vi "IR ini file file Read.vi"(2 "configuration file path":path, 11 "error in (no error) 2":errorcluster) -> (3 "IR Voltage":dbl, 4 "Ramp Time":dbl, 6 "IR LO SET resistance value(M£[)":u16=2 min=1 max=9999, 8 "IR Time":dbl, 10 "IR HI SET resistance value(M£[)":u16=9999 min=2 max=9999, 15 "error in (no error) 3":errorcluster)   [LabVIEW 2021]
uses:
  Template/Main_VI/Control/Ini.ctl
panel:
  # "M£["
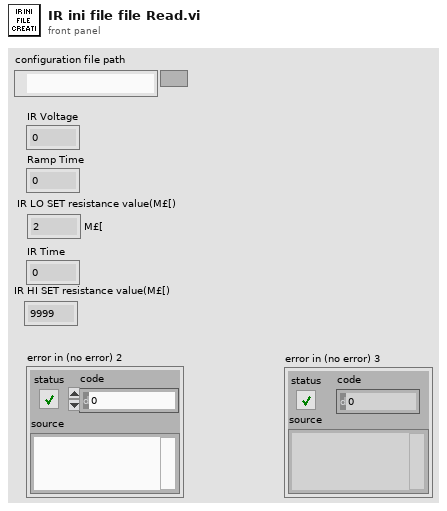
[diagram p1: front panel]
types:
  T1 = typedef "Ini.ctl" = enum16{"Write", "Read"}
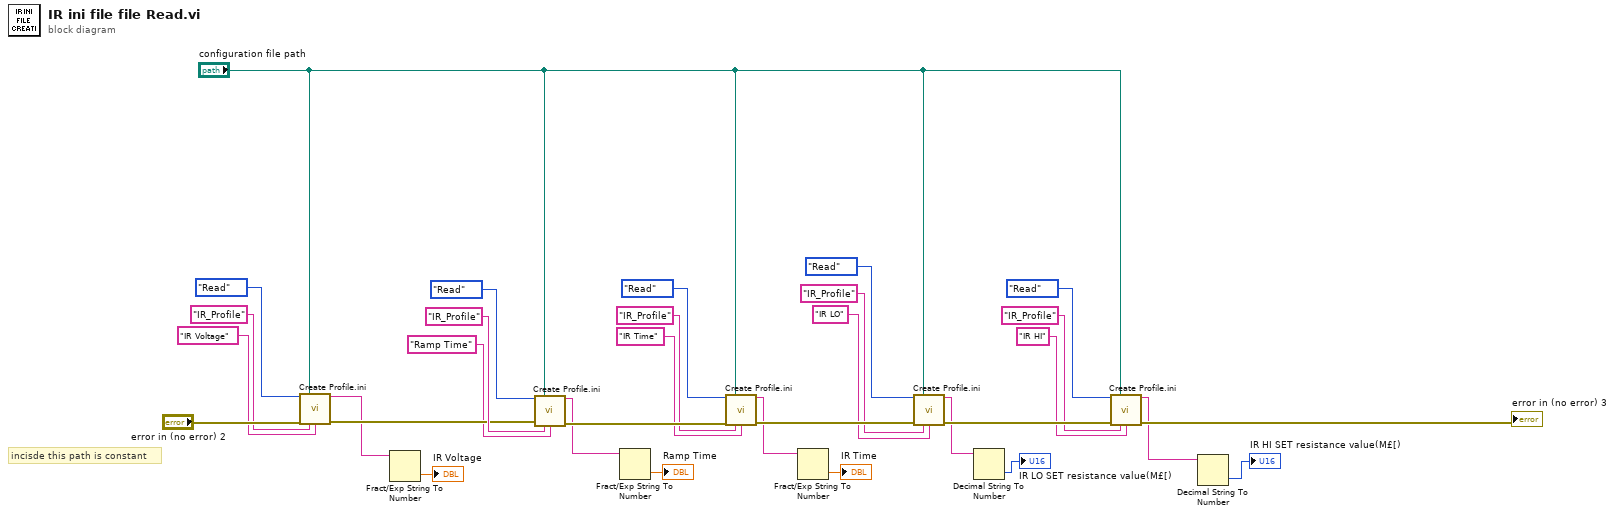
[diagram p0: block diagram]
diagram:
  # "incisde this path is constant"
  n1 = call "Create Profile.ini.vi"(0:Ini."Read", "configuration file path"="configuration file path", "error in (no error)"="error in (no error) 2", "Read Section"="IR_Profile" ("Write Section"), "Read Key"="IR Voltage" ("Write key")) -> ("value"=w12:string, "error in (no error) 3"=w20:errorcluster)  [unwired: 9 in]
  n2 = Fract/Exp String To Number(string=w12) -> (number=→"IR Voltage":dbl)  [unwired: 3 in, 1 out]
  n3 = call "Create Profile.ini.vi"(0:Ini."Read", "configuration file path"="configuration file path", "error in (no error)"=w20, "Read Section"="IR_Profile" ("Write Section"), "Read Key"="Ramp Time" ("Write key")) -> ("value"=w11:string, "error in (no error) 3"=w27:errorcluster)  [unwired: 9 in]
  n4 = Fract/Exp String To Number(string=w11) -> (number=→"Ramp Time":dbl)  [unwired: 3 in, 1 out]
  n5 = call "Create Profile.ini.vi"(0:Ini."Read", "configuration file path"="configuration file path", "error in (no error)"=w27, "Read Section"="IR_Profile" ("Write Section"), "Read Key"="IR Time" ("Write key")) -> ("value"=w10:string, "error in (no error) 3"=w26:errorcluster)  [unwired: 9 in]
  n6 = Fract/Exp String To Number(string=w10) -> (number=→"IR Time":dbl)  [unwired: 3 in, 1 out]
  n7 = call "Create Profile.ini.vi"(0:Ini."Read", "configuration file path"="configuration file path", "error in (no error)"=w26, "Read Section"="IR_Profile" ("Write Section"), "Read Key"="IR LO" ("Write key")) -> ("value"=w4:string, "error in (no error) 3"=w25:errorcluster)  [unwired: 9 in]
  n8 = Decimal String To Number(string=w4) -> (number=→"IR LO SET resistance value(M£[)":i32)  [unwired: 2 in, 1 out]
  n9 = call "Create Profile.ini.vi"(0:Ini."Read", "configuration file path"="configuration file path", "error in (no error)"=w25, "Read Section"="IR_Profile" ("Write Section"), "Read Key"="IR HI" ("Write key")) -> ("value"=w3:string, "error in (no error) 3"=→"error in (no error) 3":errorcluster)  [unwired: 9 in]
  n10 = Decimal String To Number(string=w3) -> (number=→"IR HI SET resistance value(M£[)":i32)  [unwired: 2 in, 1 out]
